vi "Initialize data structure.vi"() -> (4 "Array 2":string[](array[string]), 6 "Array":string[](array[string]), 7 "数据结构组":T1[](array[typedef]), 8 "deleted portion":string[](array[string]))   [LabVIEW 2025]
uses:
  <vilib>/Utility/file.llb/Read Delimited Spreadsheet (string).vi
  data structure.ctl
  Global_SKM.vi
panel:
  out "array w/ subset deleted":string[][](array[string])
  out "all rows":string[][](array[string])
  out "appended path":path
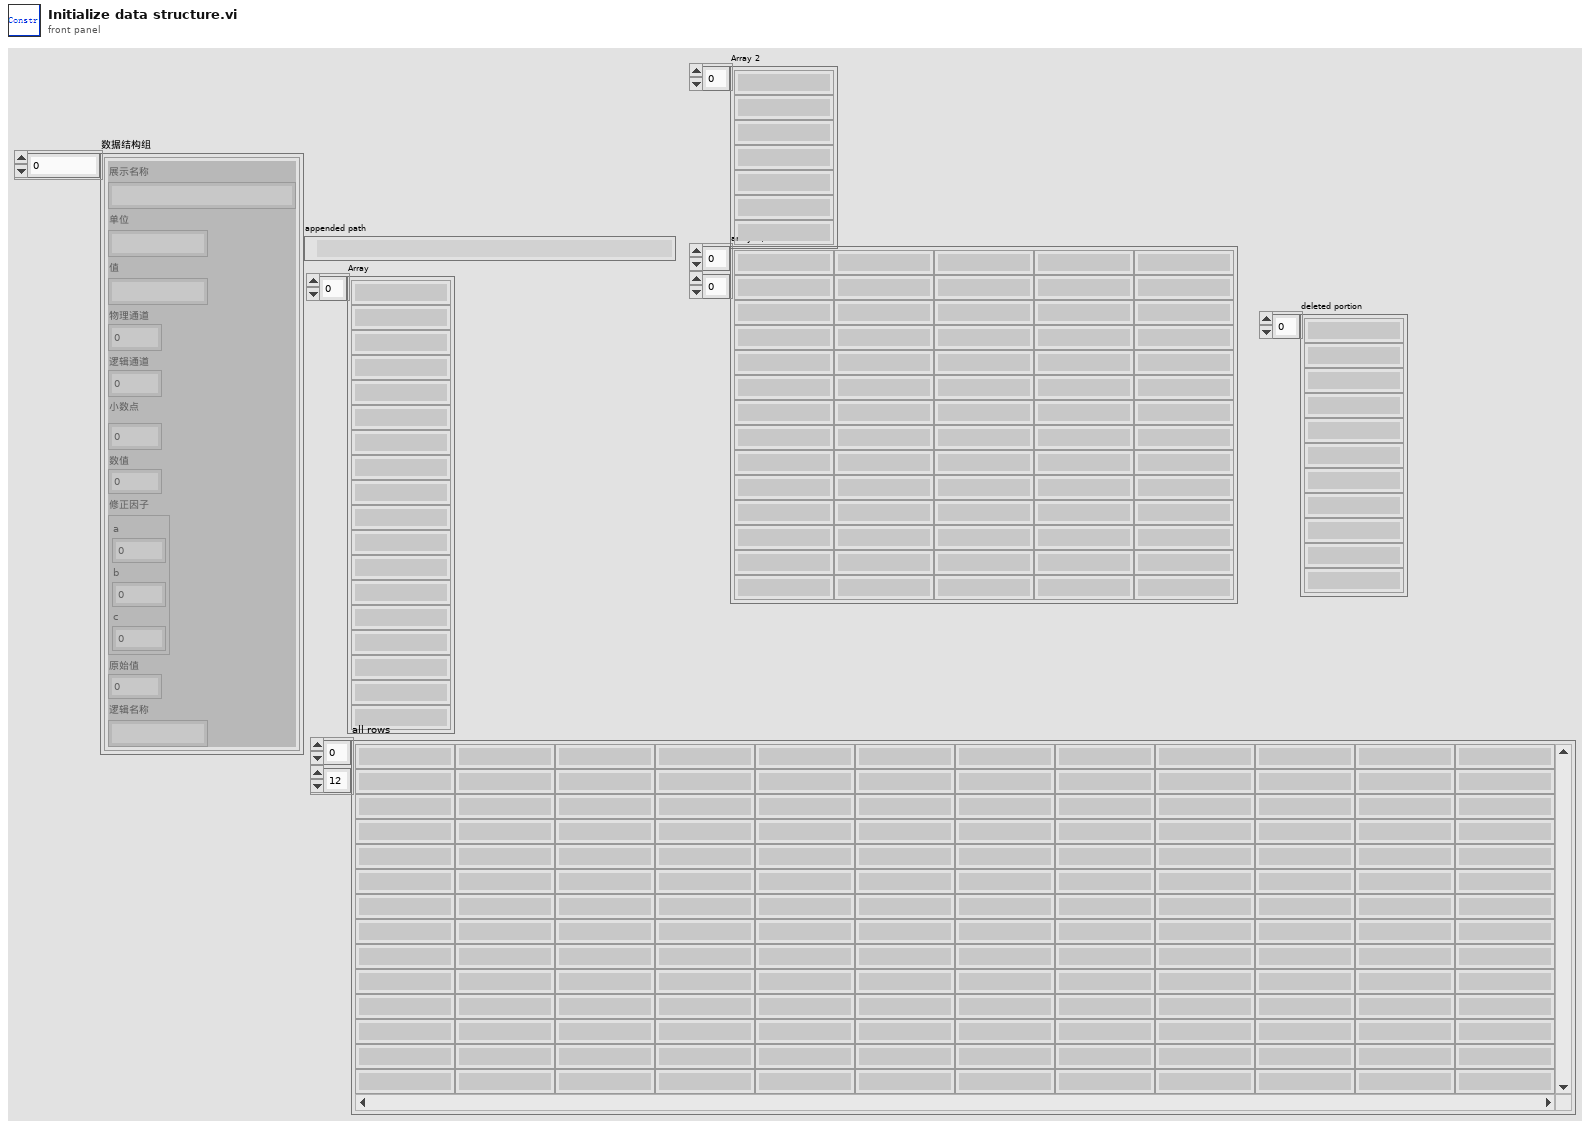
[diagram p1: front panel]
types:
  T1 = typedef "data structure.ctl" = cluster{"展示名称":string, "单位":string, "值":string, "物理通道":i32, "逻辑通道":i32, "小数点":i16, "数值":dbl, "修正因子":cluster{"a":dbl, "b":dbl, "c":dbl}, "原始值":sgl, "逻辑名称":string}
  T2 = typedef "Working condition setting_SKM.ctl" = cluster{"Test Type":u16, "FM":dbl, "Eva Power":dbl, "Comp Power":dbl, "Cond Power":dbl, "Dis Pre":string[], "Suc Pre":string[], "Dis Tem":string[], "Suc Tem":string[], "Liquid Tem":string[], "Oil Pre":string[], "Leaving Air Temp":string[], "Liquid Pre":string[], "Tested Unit Outlet Dry Temp":string[], "Compressor Temp":string[], "Evap.Leaving Temp":string[], "Evap.Entering Temp":string[], "25TR SP Choose1":string[], "25TR SP Choose2":string[], "25TR Temp Choose2":string[], "25TR Temp Choose":string[], "Ref Type":string, "Left Chamber Selected":u16, "OD Dry Temp":string[], "OD Wet Temp":string[], "OD RH":string[]}
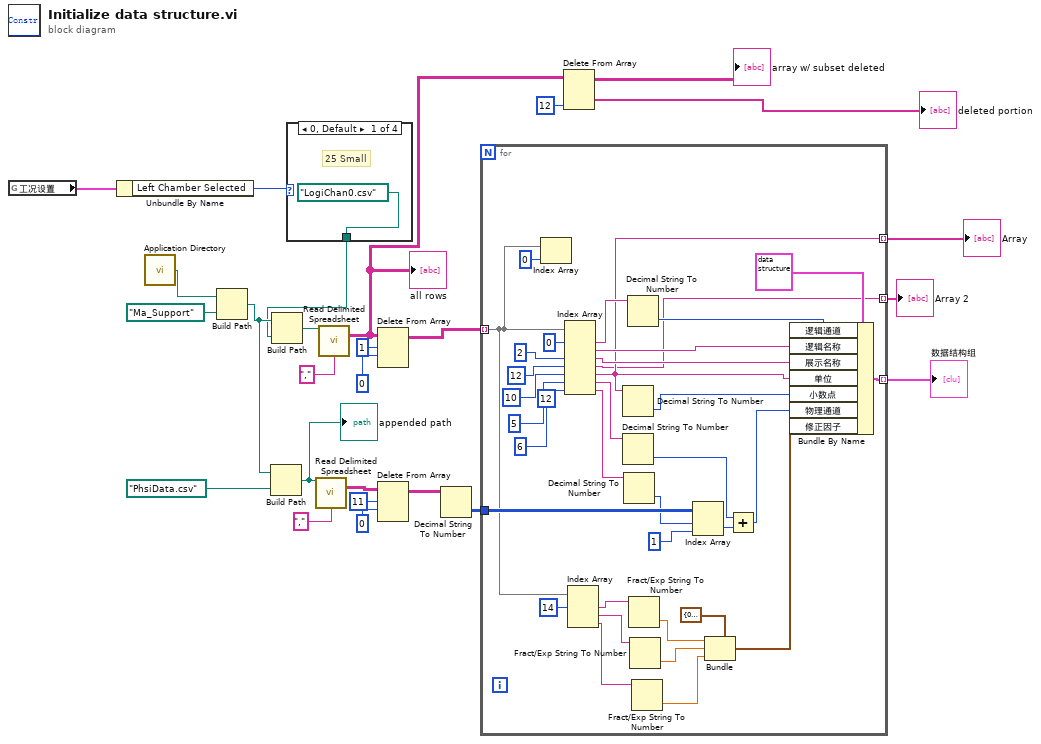
[diagram p0: block diagram]
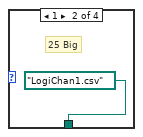
[diagram p2: hidden frame]
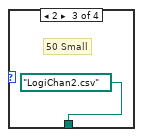
[diagram p3: hidden frame]
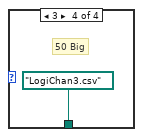
[diagram p4: hidden frame]
diagram:
  n1 = global read "Global_SKM.vi" "工况设置"() -> (w10:T2)
  n2 = Unbundle By Name(w10) -> ("Left Chamber Selected"=w9:u16)
  n3 = call <vilib>:"Application Directory.vi"() -> ("Application Directory"=w26:path)
  n4 = Build Path(base path=w26, name or relative path=path "Ma_Support" ("名称或相对路径")) -> (appended path=w19:path)
  n5 = Build Path(base path=w19, name or relative path=path "PhsiData.csv" ("名称或相对路径")) -> (appended path=w7:path)
  "appended path" <- w7
  n6 = case shown="0, Default" w9 {
    tunnel: [path "LogiChan0.csv" ("名称或相对路径") path "LogiChan1.csv" ("名称或相对路径") path "LogiChan2.csv" ("名称或相对路径") path "LogiChan3.csv" ("名称或相对路径")] -> w8
    frame 0, Default {
      # "25 Small"
    }
    frame 1 {
      # "25 Big"
    }
    frame 2 {
      # "50 Small"
    }
    frame 3 {
      # "50 Big"
    }
  }
  n7 = Build Path(base path=w19, name or relative path=w8) -> (appended path=w24:path)
  n8 = call-poly <vilib>:"Read Delimited Spreadsheet.vi"("file path (dialog if empty)"=w7, "delimiter (\\t)"="," ("delimiter (\\t)")) -> ("all rows"=w15:string[][])  [unwired: 8 in, 5 out]
  n9 = call-poly <vilib>:"Read Delimited Spreadsheet.vi"("file path (dialog if empty)"=w24, "delimiter (\\t)"="," ("delimiter (\\t)")) -> ("all rows"=w5:string[][])  [unwired: 8 in, 5 out]
  "all rows" <- w5
  n10 = Delete From Array(array=w5, length=1 ("长度"), index (row)=0 ("索引 (行)")) -> (array with subset deleted=w20:string[][])  [unwired: 1 in, 1 out]
  n11 = Delete From Array(array=w15, length=11 ("长度"), index (row)=0 ("索引 (行)")) -> (array with subset deleted=w13:string[][])  [unwired: 1 in, 1 out]
  n12 = Decimal String To Number(string=w13) -> (number=w12:i32[][])  [unwired: 2 in, 1 out]
  n13 = for {
    tunnel: w20 -> [w34] mode=indexing
    tunnel: w12 -> [w55]
    tunnel: [w49] -> w11 mode=indexing
    tunnel: [w32] -> w6 mode=indexing
    tunnel: [w31] -> w1 mode=indexing
    (unwired) 12 ("index")
    n14 = Index Array(array=w34, index=0) -> ()  [unwired: 1 out]
    n15 = Index Array(array=w34, index #1=0 ("索引"), index #3=2 ("索引"), index #4=12 ("索引"), index #5=10 ("索引"), index #6=5 ("索引"), index #7=6 ("索引")) -> (element #1=w37:string, element #2=w35:string, element #3=w62:string, element #4=w31:string, element #5=w32:string, element #6=w57:string, element #7=w56:string)  [unwired: 1 in]
    n16 = Index Array(array=w34, index #1=14 ("索引")) -> (element #1=w46:string, element #2=w45:string, element #3=w44:string)  [unwired: 2 in]
    n17 = Decimal String To Number(string=w32) -> (number=w48:i32)  [unwired: 2 in, 1 out]
    n18 = Decimal String To Number(string=w57) -> (number=w52:i32)  [unwired: 2 in, 1 out]
    n19 = Decimal String To Number(string=w56) -> (number=w54:i32)  [unwired: 2 in, 1 out]
    n20 = Decimal String To Number(string=w37) -> (number=w36:i32)  [unwired: 2 in, 1 out]
    n21 = Fract/Exp String To Number(string=w46) -> (number=w42:dbl)  [unwired: 3 in, 1 out]
    n22 = Fract/Exp String To Number(string=w45) -> (number=w41:dbl)  [unwired: 3 in, 1 out]
    n23 = Fract/Exp String To Number(string=w44) -> (number=w40:dbl)  [unwired: 3 in, 1 out]
    n24 = Index Array(array=w55, index (row)=w54, index (col)=1 ("禁用的索引 (列)")) -> (element=w51:i32)
    n25 = Bundle(cluster=cluster{"a":dbl, "b":dbl, "c":dbl} {"a"=0.0, "b"=0.0, "c"=0.0} ("修正因子"), "a"=w42, "b"=w41, "c"=w40) -> (w39:cluster{"a":dbl, "b":dbl, "c":dbl})
    n26 = Add(x=w52, y=w51) -> (x+y=w50:i32)
    n27 = Bundle By Name(cluster=T1 {"展示名称"="", "单位"="", "值"="", "物理通道"=0, "逻辑通道"=0, "小数点"=0, "数值"=0.0, "修正因子"={"a"=0.0, "b"=0.0, "c"=0.0}, "原始值"=0.0, "逻辑名称"=""} ("数据结构"), "逻辑通道"=w36, "逻辑名称"=w35, "展示名称"=w62, "单位"=w32, "小数点"=w48, "物理通道"=w50, "修正因子"=w39) -> (w49:T1)
  }
  "数据结构组" <- w11
  "Array" <- w6
  "Array 2" <- w1
  n28 = Delete From Array(array=w5, index (col)=12 ("disabled index (col)")) -> (deleted portion=→"deleted portion":string[], array with subset deleted=→"array w/ subset deleted":string[][])  [unwired: 2 in]
